vi "Run.vi"(8 "error in (no error)":errorcluster, 10 "UI Refs":T1, 11 "3way Lap":refnum<class "3way Lap.lvclass">) -> (0 "error out":errorcluster, 3 "3way Lap out":refnum<class "3way Lap.lvclass">)   [LabVIEW 2025, in "Flow Grind.lvlib" / "3way Lap.lvclass"]
uses:
  3way Lap.lvclass
  3way Lap.lvclass/3way Lap.ctl
  Users/Public/Documents/Sandia National Labs/TSS Plugin/Tests/XY Plotter.lvlibp/XY  Plotter/XY Plotter.lvclass
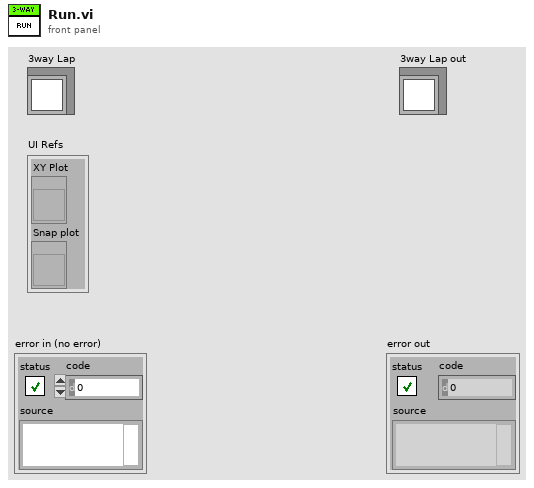
[diagram p1: front panel]
types:
  T1 = cluster{"XY Plot":refnum<vi>, "Snap plot":refnum<vi>}
  T2 = cluster{"Name":string, "Color":u32, "Style":u8, "Point Style":u8, "Name Visible":bool, "Allow Drag":bool, "Annotation Mode":u32, "Plot":i32, "Index":i32, "Position":cluster{"X":dbl, "Y":dbl}, "X Scale":u32, "Y Scale":u32, "Show Arrow":bool, "Lock Name":bool, "Plot Area":i32, "Label Offset":cluster{"X":dbl, "Y":dbl}}
  T3 = typedef "LVAnnotationListTypeDef.ctl" = cluster{"Name":string, "Color":u32, "Style":u8, "Point Style":u8, "Name Visible":bool, "Allow Drag":bool, "Annotation Mode":u32, "Plot":i32, "Index":i32, "Position":cluster{"X":dbl, "Y":dbl}, "X Scale":u32, "Y Scale":u32, "Show Arrow":bool, "Lock Name":bool, "Plot Area":i32, "Label Offset":cluster{"X":dbl, "Y":dbl}}[]
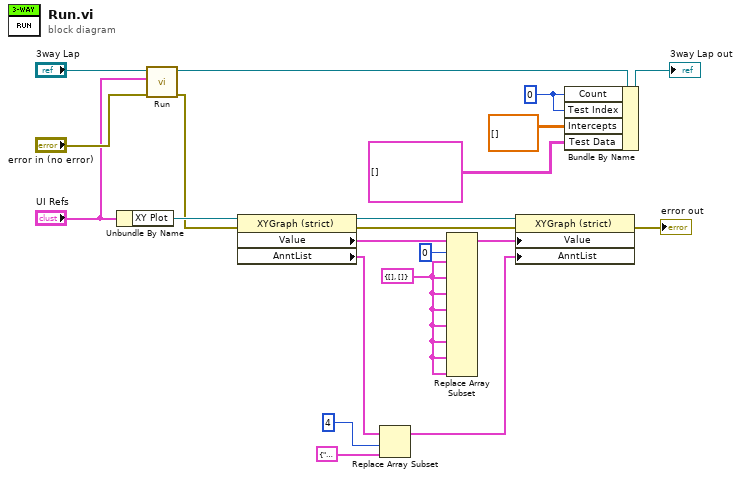
[diagram p0: block diagram]
diagram:
  w7 = cluster{"Wavenumber":dbl[], "Data":dbl[]} {"Wavenumber"=[], "Data"=[]} ("Spectrum")
  w15 = 0 ("Count")
  n1 = Unbundle By Name("UI Refs") -> ("XY Plot"=w14:refnum<vi>)
  n2 = call-parent "Run.vi"("error in (no error)"="error in (no error)", "UI Refs"="UI Refs", "XY Plotter"="3way Lap") -> ("error out"=w13:errorcluster, "XY Plotter out"=w18:refnum<class "3way Lap.lvclass">)  [unwired: 7 in]
  n3 = property class="XYGraph (strict)"(reference=w14) -> (reference out=w11:refnum<vi>, "Value"=w10:cluster{"Wavenumber":dbl[], "Data":dbl[]}[], "AnntList"=w6:T3)  [unwired: 1 in, 1 out]
  n4 = Replace Array Subset(array=w6, new element=T2 {"Name"="", "Color"=0, "Style"=0, "Point Style"=0, "Name Visible"=FALSE, "Allow Drag"=FALSE, "Annotation Mode"=0, "Plot"=0, "Index"=0, "Position"={"X"=0.0, "Y"=0.0}, "X Scale"=0, "Y Scale"=0, "Show Arrow"=FALSE, "Lock Name"=FALSE, "Plot Area"=0, "Label Offset"={"X"=0.0, "Y"=0.0}} ("new element/subarray"), index=4) -> (w5:T3)
  n5 = Replace Array Subset(array=w10, new element #1=w7, index #1=0 ("index"), new element #2=w7, new element #3=w7, new element #4=w7, new element #5=w7, new element #6=w7, new element #7=w7, new element #8=w7) -> (w9:cluster{"Wavenumber":dbl[], "Data":dbl[]}[])  [unwired: 7 in]
  n6 = property class="XYGraph (strict)"(reference=w11, error in=w13, "Value"=w9, "AnntList"=w5) -> (error out=→"error out":errorcluster)  [unwired: 1 out]
  n7 = Bundle By Name(cluster=w18, "Count"=w15, "Test Index"=w15, "Intercepts"=dbl[][] [], "Test Data"=cluster{"Best Linear Fit":dbl[], "Y":dbl[]}[][] []) -> (→"3way Lap out":refnum<class "3way Lap.lvclass">)
